vi "piano.vi"() -> ()   [LabVIEW 2018]
uses:
  <vilib>/measure/NI_MABase.lvlib
panel:
  in  "?":bool
  in  "SA":bool
  in  "NI":bool
  in  "DHA":bool
  in  "PA":bool
  in  "MA":bool
  in  "GA":bool
  in  "RE":bool
  in  "SA":bool
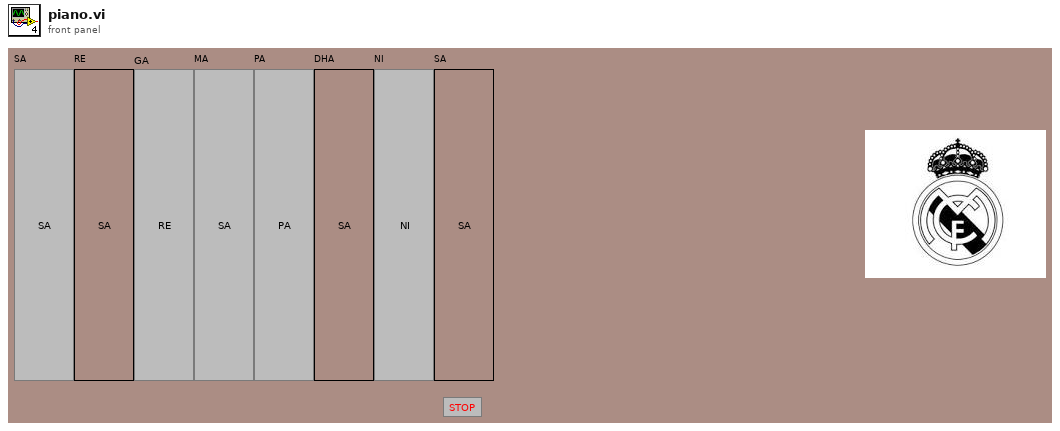
[diagram p1: front panel]
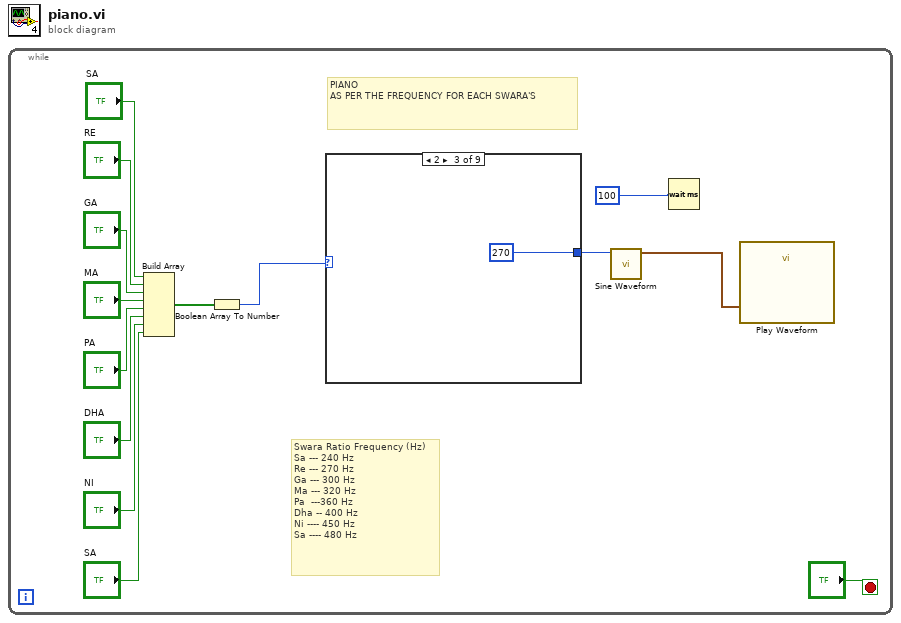
[diagram p0: block diagram]
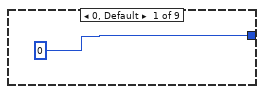
[diagram p2: hidden frame]
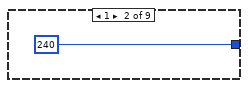
[diagram p3: hidden frame]
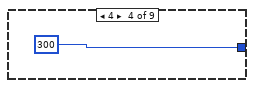
[diagram p4: hidden frame]
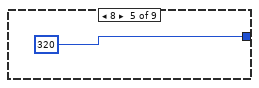
[diagram p5: hidden frame]
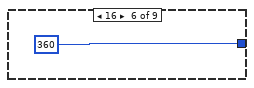
[diagram p6: hidden frame]
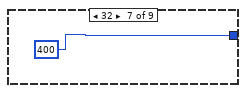
[diagram p7: hidden frame]
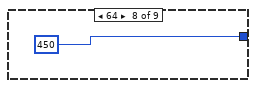
[diagram p8: hidden frame]
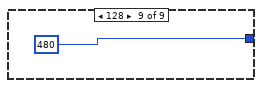
[diagram p9: hidden frame]
diagram:
  n1 = while {
    stop <- "?" stop-if-true
    # "PIANO \nAS PER THE FREQUENCY FOR EACH SWARA'S"
    # "Swara\tRatio\tFrequency (Hz)\nSa\t---\t240 Hz\nRe ---\t270 Hz\nGa ---\t300 Hz\nMa ---\t320 Hz\nPa \t---360 Hz\nDha --\t400 Hz\nNi ----\t450 Hz\nSa ----\t480 Hz"
    n2 = Build Array "Build Array"("SA", "RE", "GA", "MA", "PA", "DHA", "NI", "SA") -> (w10:bool[])
    n3 = Boolean Array To Number(Boolean array=w10) -> (number=w4:u32)
    n4 = case shown="2" w4 {
      tunnel: [0 240 270 300 320 360 400 450 480] -> w5
      frame 0, Default {
      }
      frame 1 {
      }
      frame 2 {
      }
      frame 4 {
      }
      frame 8 {
      }
      frame 16 {
      }
      frame 32 {
      }
      frame 64 {
      }
      frame 128 {
      }
    }
    n5 = call <vilib>:"Sine Waveform.vi"("frequency"=w5) -> ("signal out"=w1:waveform(dbl))  [unwired: 9 in, 1 out]
    n6 = Wait (ms)(milliseconds to wait=100) -> ()  [unwired: 1 out]
    n7 = call "Play Waveform"("Data"=w1) -> ()  [unwired: 18 in, 1 out]
  }
